vi "Generate Status-API Mapping mermaid.vi"(8 "Error in":errorcluster caption="Error in (no error)") -> (0 "Error out":errorcluster, 2 "Array":T1(array[cluster]), 3 "String":string)   [LabVIEW 2020, in "CSM Mermaid Support.lvlib"]
uses:
  CSM Mermaid Support.lvlib
  <userlib>/_NEVSTOP/Communicable State Machine(CSM)/Communicable State Machine.lvlib
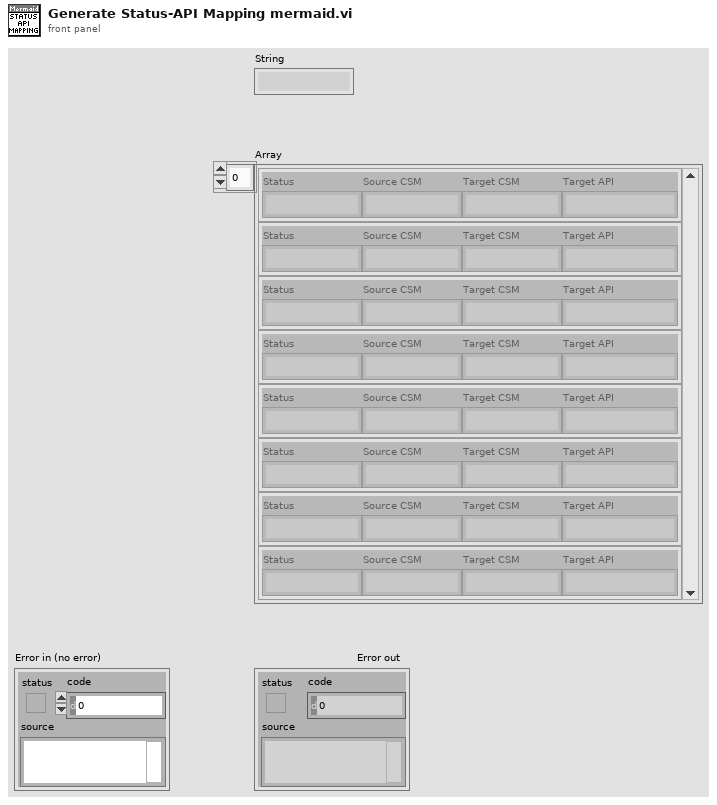
[diagram p1: front panel]
types:
  T1 = cluster{"Status":string, "Source CSM":string, "Target CSM":string, "Target API":string}[]
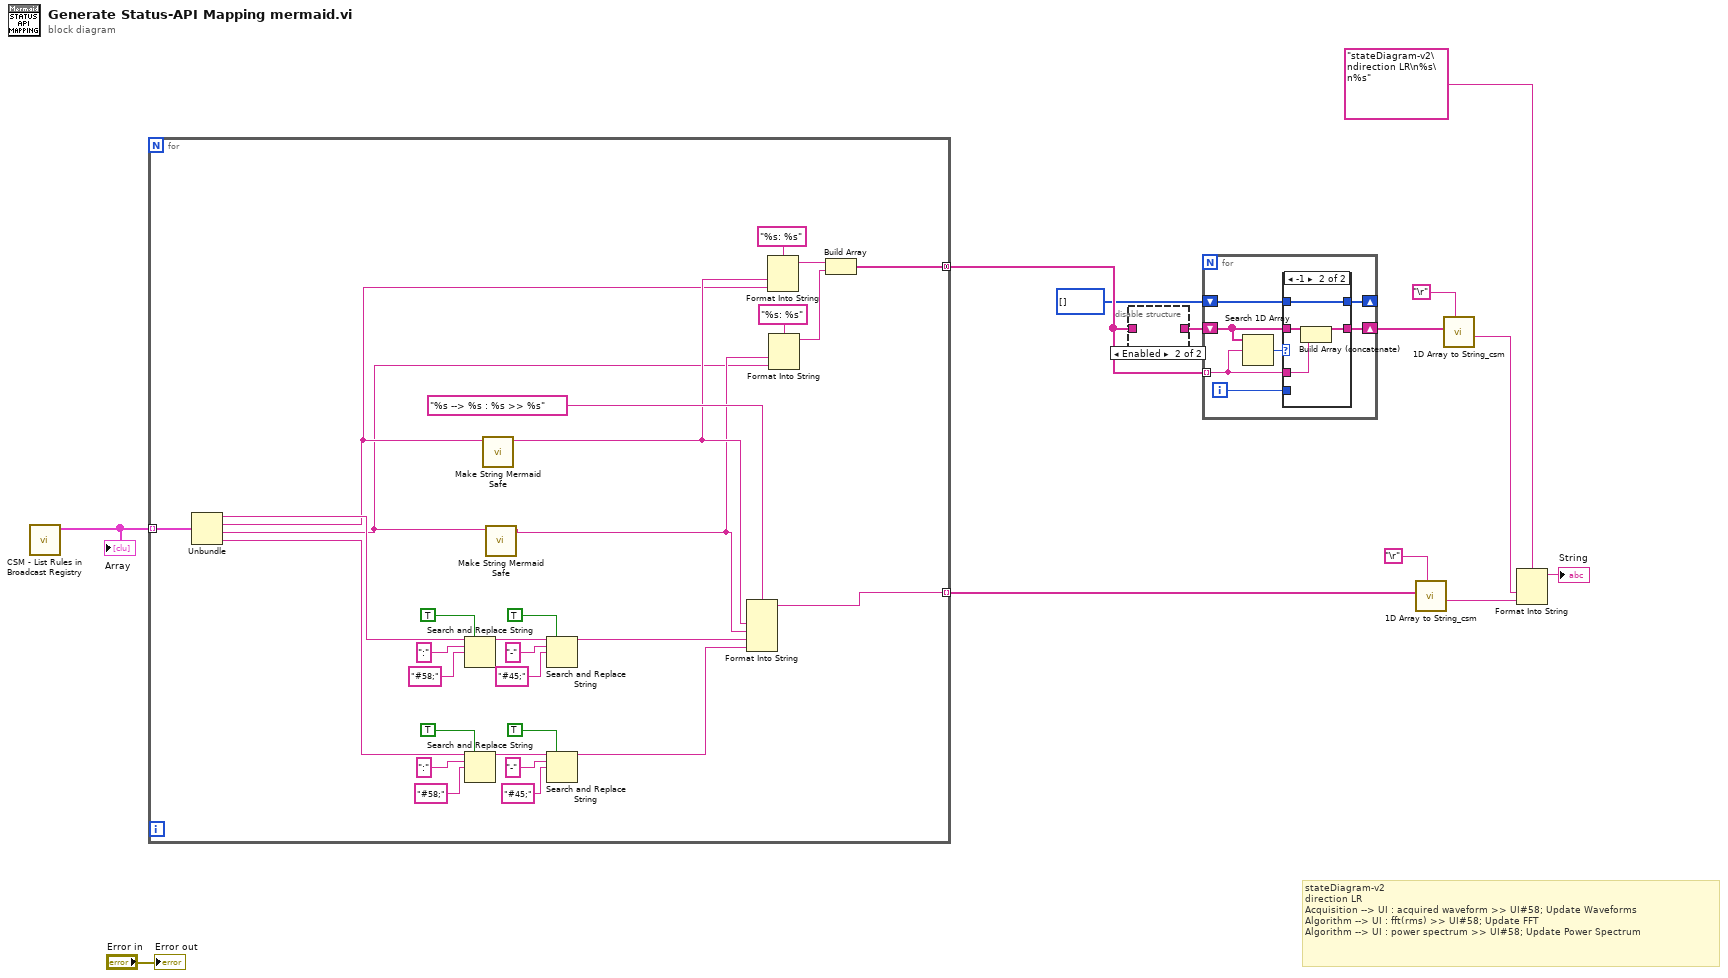
[diagram p0: block diagram]
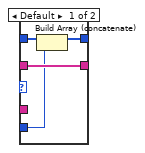
[diagram p3: hidden frame]
diagram:
  # "stateDiagram-v2\ndirection LR\nAcquisition --> UI : acquired waveform >> UI#58; Update Waveforms\nAlgorithm --> UI : fft(rms) >> UI#58; Update FFT\nAlgorithm --> UI : power spectrum >> UI#58; Update Power Spectrum"
  n1 = call <userlib>:"CSM - List Rules in Broadcast Registry.vi"() -> ("Entries"=w1:T1)  [unwired: 10 in, 1 out]
  "Array" <- w1
  n2 = for {
    tunnel: w1 -> [w43] mode=indexing
    tunnel: [w41] -> w11 mode=indexing
    tunnel: [w16] -> w7 mode=concatenating
    n3 = Unbundle(w43) -> ("Status"=w25:string, "Source CSM"=w19:string, "Target CSM"=w14:string, "Target API"=w37:string)
    n4 = Search and Replace String(replace all?=TRUE ("replace all? (F)"), input string=w25, search string=":", replace string="#58;" ("search string")) -> (result string=w26:string)  [unwired: 4 in, 3 out]
    n5 = Search and Replace String(replace all?=TRUE ("replace all? (F)"), input string=w37, search string=":", replace string="#58;" ("search string")) -> (result string=w33:string)  [unwired: 4 in, 3 out]
    n6 = call "Make String Mermaid Safe.vi"("Source CSM"=w19) -> ("result string"=w20:string)  [unwired: 10 in]
    n7 = call "Make String Mermaid Safe.vi"("Source CSM"=w14) -> ("result string"=w15:string)  [unwired: 10 in]
    n8 = Search and Replace String(replace all?=TRUE ("replace all? (F)"), input string=w26, search string="-", replace string="#45;" ("search string")) -> (result string=w24:string)  [unwired: 4 in, 3 out]
    n9 = Search and Replace String(replace all?=TRUE ("replace all? (F)"), input string=w33, search string="-", replace string="#45;" ("search string")) -> (result string=w23:string)  [unwired: 4 in, 3 out]
    n10 = Format Into String(format string="%s --> %s : %s >> %s", w20, w15, w24, w23) -> (resulting string=w41:string)  [unwired: 2 in, 1 out]
    n11 = Format Into String(format string="%s: %s", w20, w19) -> (resulting string=w18:string)  [unwired: 2 in, 1 out]
    n12 = Format Into String(format string="%s: %s", w15, w14) -> (resulting string=w17:string)  [unwired: 2 in, 1 out]
    n13 = Build Array(w18, w17) -> (w16:string[])
  }
  n14 = disable-structure shown="Enabled" {
    disable-tunnel: [w44 _] -> w3
    disable-tunnel: w7 -> [w44 _]
    frame Disabled {
    }
    frame Enabled {
    }
  }
  n15 = for {
    tunnel: w7 -> [w50] mode=indexing
    shift-right: [w49] -> w5
    shift-left: w3 -> [w48]
    shift-right: [w46] -> _
    shift-left: i32[] [] -> [w45]
    i -> [w47]
    n16 = Search 1D Array(1D array=w48, element=w50) -> (index of element=w51:i32)  [unwired: 1 in]
    n17 = case shown="-1" w51 {
      tunnel: w50 -> [_ w59]
      tunnel: [w55 w57] -> w49
      tunnel: w48 -> [w55 w58]
      tunnel: w47 -> [w52 _]
      tunnel: [w53 w56] -> w46
      tunnel: w45 -> [w54 w56]
      frame Default {
        n18 = Build Array (concatenate)(w54, w52) -> (w53:i32[])
      }
      frame -1 {
        n19 = Build Array (concatenate)(w58, w59) -> (w57:string[])
      }
    }
  }
  n20 = call <userlib>:"1D Array to String_csm.vi"("delimiter (Tab)"="\r", "Array of Strings"=w11) -> ("delimited string"=w10:string)  [unwired: 9 in]
  n21 = call <userlib>:"1D Array to String_csm.vi"("delimiter (Tab)"="\r", "Array of Strings"=w5) -> ("delimited string"=w4:string)  [unwired: 9 in]
  n22 = Format Into String(format string="stateDiagram-v2\ndirection LR\n%s\n%s", w4, w10) -> (resulting string=→"String":string)  [unwired: 2 in, 1 out]
  "Error out" <- "Error in"
